vi "1_Power_Transmission_Line_Fault_Classification(Training).vi"() -> ()   [LabVIEW 2020]
uses:
  <vilib>/Ngene/Deep Learning Toolkit/Toolkit/NN_Train/Controls/NN_LR_Policy_Cfg.ctl
  <vilib>/Ngene/Deep Learning Toolkit/Toolkit/NN_Train/Controls/NN_LR_Policy_Type.ctl
  <vilib>/Ngene/Deep Learning Toolkit/Toolkit/NN_Train/Controls/NN_Train_Session_Data.ctl
  <vilib>/Ngene/Deep Learning Toolkit/Toolkit/NN_Train/Controls/NN_Train_Params.ctl
  <vilib>/Ngene/Deep Learning Toolkit/Toolkit/NN_Train/Controls/NN_Train_Optimizer.ctl
  <vilib>/Ngene/Deep Learning Toolkit/Toolkit/NN_Train/Controls/NN_Train_Data_Sampling.ctl
  <vilib>/Ngene/Deep Learning Toolkit/Toolkit/NN_Network/Controls/NN_Device.ctl
  <vilib>/Ngene/Deep Learning Toolkit/Toolkit/NN_Layers/Layers/Input/Controls/NN_Layer_Config(Input1D).ctl
  <vilib>/Ngene/Deep Learning Toolkit/Toolkit/NN_Data/Controls/NN_Data_type.ctl
  <vilib>/Ngene/Deep Learning Toolkit/Toolkit/NN_Layers/Layers/FC/Controls/NN_Layer_Config(FC).ctl
  <vilib>/Ngene/Deep Learning Toolkit/Toolkit/NN_Layers/Layers/BatchNorm/Controls/NN_BN_Params.ctl
  <vilib>/Ngene/Deep Learning Toolkit/Toolkit/NN_Activations/Controls/NN_Activation_Type.ctl
  <vilib>/Ngene/Deep Learning Toolkit/Toolkit/NN_Layers/Controls/NN_Layer_Init_Params.ctl
  <vilib>/Ngene/Deep Learning Toolkit/Toolkit/NN_Layers/Controls/NN_Layer_Weight_Init_Type.ctl
  <vilib>/Ngene/Deep Learning Toolkit/Toolkit/NN_Network/Controls/NN_Save_Before_Destroy_Options.ctl
  <vilib>/Ngene/Deep Learning Toolkit/Toolkit/NN_Layers/Layers/DropOut3D/Controls/NN_Layer_Config(DropOut3D).ctl
  <vilib>/Ngene/Deep Learning Toolkit/Toolkit/NN_Layers/Layers/FC/NN_Layer_Create(FC).vi
  <vilib>/Ngene/Deep Learning Toolkit/Toolkit/NN_Layers/Layers/Dropout/NN_Layer_Create(DropOut).vi
  <vilib>/Ngene/Deep Learning Toolkit/Toolkit/NN_Layers/Layers/Input/NN_Layer_Create(Input1D).vi
  <vilib>/Ngene/Deep Learning Toolkit/Toolkit/NN_Train/Eval_Loss/NN_Calc_Cofusion_Matrix/NN_Calc_Confusion_Matrix(In1D_Out1D).vi
  <vilib>/Ngene/Deep Learning Toolkit/Toolkit/NN_Train/Loss_Functions/NN_Set_Loss(CrossEntropy).vi
  <vilib>/Ngene/Deep Learning Toolkit/Toolkit/NN_Train/Eval_Loss/NN_Eval_Test_Error_Loss/NN_Eval(In1D_Out1D).vi
  <vilib>/Ngene/Deep Learning Toolkit/Toolkit/NN_Network/subVIs/NN_Predict/NN_Predict(In1D_Out1D).vi
  <vilib>/Ngene/Deep Learning Toolkit/Toolkit/NN_Layers/Layers/SoftMax/NN_Layer_Create(SoftMax).vi
  <vilib>/Ngene/Deep Learning Toolkit/Toolkit/Deep_Learning_Toolkit_by_Ngene.lvlib
  <vilib>/ptbypt/NI_PtbyPt.lvlib
panel:
  in  "Tab Control":enum32{"Training", "Evaluation"}(tab)
  in  "LR Update Policy":T1={"Policy_Type"=enum."Step", "LR0"=1e-05, "k"=200.0, "WarmUp_Policy"=enum."Ramp", "WarmUp_Iter"=1000, "WarmUp_Ratio"=10.0} {"WarmUp_Ratio" min=1; "WarmUp_Iter" min=1; "LR0" format="%.7f"}
  out "Session Data":T3={"Epochs"=251.7248, "Tot_Iter"=58998, "LR"=5e-06, "LR_iter"=58999}
  in  "NN_Train_Params":T4={"Optimizer"=enum."Adam", "Beta_1"=0.9, "Beta_2"=0.999, "Weight Decay(L1)"=7e-07, "Weight Decay(L2)"=7e-07, "Data_Sampling"=enum."Random"}
  in  "Stop Training":bool
  out "Test Error":sgl=0.024555556 format="%#.6g"
  out "Test Loss":sgl=0.121348076 format="%#.6g"
  in  "NN_Device":T7=enum."GPU"
  out "Loss Graphs":cluster{"mean":dbl, "mean":dbl, "mean":dbl}(graph)={"mean"=0.14842731654644012, "mean"=0.121348075568676, "mean"=0.02455555647611618}
  in  "Eval":bool
  out "Training Loss":sgl=0.21247883 format="%#.6g"
  in  "Train dataset path":path=path "D:/Ngene/GitHub/deepltk_examples/2_Waveform_Processing/23_Power_Transmission_Line_Fault_Classification/Dataset/Train"
  in  "Test dataset path":path=path "D:/Ngene/GitHub/deepltk_examples/2_Waveform_Processing/23_Power_Transmission_Line_Fault_Classification/Dataset/Test"
  out "Time_Elapsed":dbl=138.95477960000062 format="%<%H:%M:%S>t"
  out "Confusion Matrix":string[][](table)=[["1500", "0", "0", "0", "0", "0", "1.0000"], ["0", "1492", "0", "0", "8", "0", "0.9947"], ["0", "0", "1498", "0", "0", "2", "0.9987"], ["0", "0", "0", "1423", "68", "9", "0.9487"], ["0", "0", "0", "78", "1411", "11", "0.9407"], ["0", "0", "40", "3", "2", "1455", "0.9700"], ["1.0000", "1.0000", "0.9740", "0.9461", "0.9476", "0.9851", ""]]
  # "Overview: This example demonstrates the usage of DeepLTK for solving Power Transmission Line Fault classification problem.\nRequirements: Deep Learning Toolkit for LabVIEW.\nInstructions:\n1.  Run the VI with current configuration of the training parameters and Learning Rate update policy.\n2. Observe how the training loss is decreasing.\n3. Wait about 2 minutes and press the \"Stop\" button when the loss is not decreasing anymore."
  # "Power Transmission Line Fault Classification - Training"
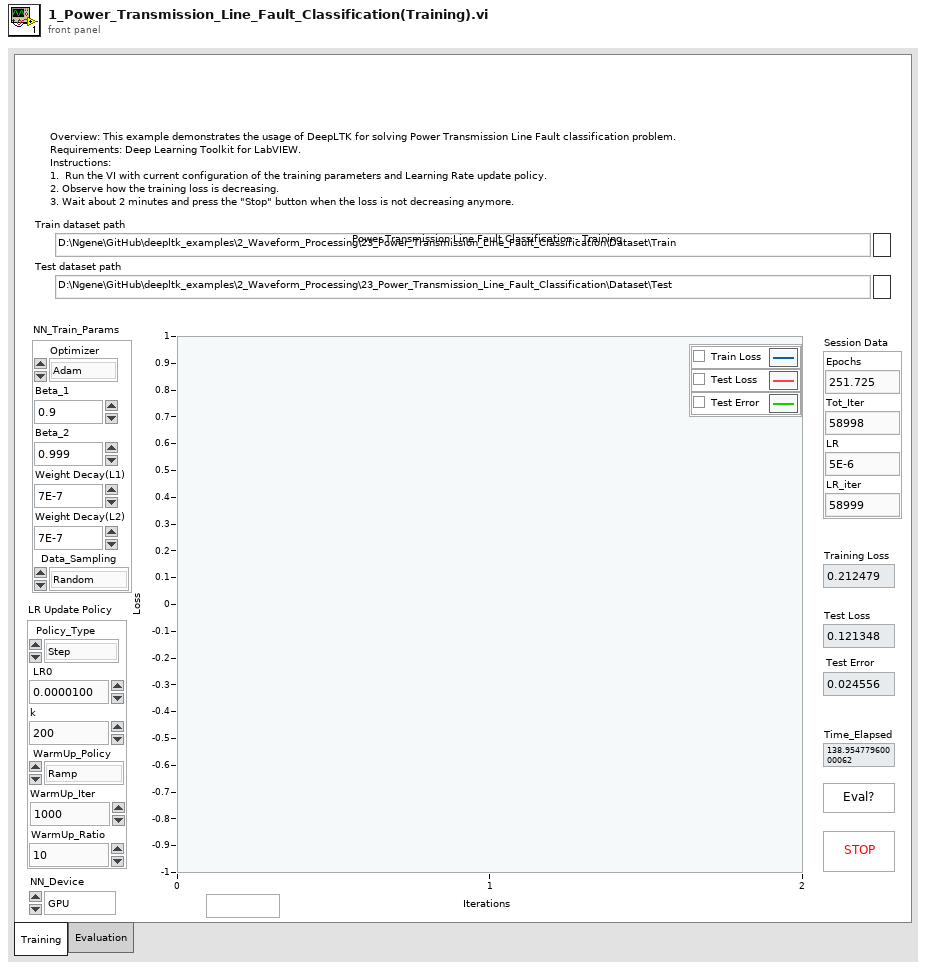
[diagram p1: front panel]
types:
  T1 = typedef "Deep_Learning_Toolkit_by_Ngene.lvlib/NN_LR_Policy_Cfg.ctl" = cluster{"Policy_Type":T2, "LR0":dbl, "k":sgl, "WarmUp_Policy":enum16{"Step", "Ramp"}, "WarmUp_Iter":i32, "WarmUp_Ratio":sgl}
  T2 = typedef "Deep_Learning_Toolkit_by_Ngene.lvlib/NN_LR_Policy_Type.ctl" = enum16{"Manual", "Step", "Exp", "1/t"}
  T3 = typedef "Deep_Learning_Toolkit_by_Ngene.lvlib/NN_Train_Session_Data.ctl" = cluster{"Epochs":sgl, "Tot_Iter":i32, "LR":sgl, "LR_iter":i32}
  T4 = typedef "Deep_Learning_Toolkit_by_Ngene.lvlib/NN_Train_Params.ctl" = cluster{"Optimizer":T5, "Beta_1":sgl, "Beta_2":sgl, "Weight Decay(L1)":sgl, "Weight Decay(L2)":sgl, "Data_Sampling":T6}
  T5 = typedef "Deep_Learning_Toolkit_by_Ngene.lvlib/NN_Train_Optimizer.ctl" = enum16{"SGD", "Adam", "Adagrad", "Adadelta", "RMSProp", "Nesterov"}
  T6 = typedef "Deep_Learning_Toolkit_by_Ngene.lvlib/NN_Train_Data_Sampling.ctl" = enum16{"Random", "Sequential"}
  T7 = typedef "Deep_Learning_Toolkit_by_Ngene.lvlib/NN_Device.ctl" = enum16{"CPU", "GPU"}
  T8 = typedef "Deep_Learning_Toolkit_by_Ngene.lvlib/NN_Layer_Config(DropOut3D).ctl" = cluster{"Name":string, "Probability":sgl}
  T9 = typedef "Deep_Learning_Toolkit_by_Ngene.lvlib/NN_Save_Before_Destroy_Options.ctl" = cluster{"CFG?":bool, "Weights?":bool, "Render?":bool}
  T10 = typedef "Deep_Learning_Toolkit_by_Ngene.lvlib/NN_Layer_Config(FC).ctl" = cluster{"Name":string, "Size":i32, "BN":bool, "BN_Params":T11, "Activation":T12, "Has Bias?":bool, "Init_Params":T13, "Custom_Params":string}
  T11 = typedef "Deep_Learning_Toolkit_by_Ngene.lvlib/NN_BN_Params.ctl" = cluster{"epsilon":sgl, "momentum":sgl}
  T12 = typedef "Deep_Learning_Toolkit_by_Ngene.lvlib/NN_Activation_Type.ctl" = enum16{"Sigmoid", "ReLU", "LReLU", "ReLU6", "GELU", "tanh", "Swish", "Mish", "None"}
  T13 = typedef "Deep_Learning_Toolkit_by_Ngene.lvlib/NN_Layer_Init_Params.ctl" = cluster{"Init_Type":T14, "Value":sgl}
  T14 = typedef "Deep_Learning_Toolkit_by_Ngene.lvlib/NN_Layer_Weight_Init_Type.ctl" = enum16{"Const", "Uniform", "Gaussian", "Xavier"}
  T15 = typedef "Deep_Learning_Toolkit_by_Ngene.lvlib/NN_Layer_Config(Input1D).ctl" = cluster{"Name":string, "Size":i32, "Data_Type":T16, "Shift":sgl, "Scale":sgl}
  T16 = typedef "Deep_Learning_Toolkit_by_Ngene.lvlib/NN_Data_type.ctl" = enum16{"I8", "U8", "I16", "U16", "U32 ARGB", "SGL"}
  T17 = typedef "Deep_Learning_Toolkit_by_Ngene.lvlib/NN_DataSets_All(In1D_Out1D).ctl" = cluster{"Train":T18, "Validation":T18, "Test":T18}
  T18 = typedef "Deep_Learning_Toolkit_by_Ngene.lvlib/NN_DataSet(In1D_Out1D).ctl" = cluster{"Inputs Ref.":variant, "Outputs Ref.":T19, "Dims_In":i32, "Dataset_Size":i32, "Dims_Out":i32, "Labels":string[], "File Paths":path[], "Custom_Data":variant}
  T19 = typedef "Deep_Learning_Toolkit_by_Ngene.lvlib/NN_Data_ref(2D_SGL).ctl" = refnum<data-value>
  T20 = typedef "Deep_Learning_Toolkit_by_Ngene.lvlib/NN.ctl" = cluster{"Name":string, "No of Layers":i32, "mBatch":i32, "Layers":T21[], "Dimty":T22, "Dims_In":T23, "Dims_Out":T23, "Working_Dir":path, "Train?":bool, "Train_Params":T4, "LR_Update_Policy":T1, "Session Data":T3, "Ground_truth":T24, "NNg_hdls":T25, "NN_Device":T7, "GPU Id":i32, "Labels":string[], "Loss_Type":T26, "Loss_Cfg_Prms":variant, "NNG_WS":T27, "DryRun?":bool}
  T21 = typedef "Deep_Learning_Toolkit_by_Ngene.lvlib/NN_Layer_ref.ctl" = refnum<file>
  T22 = typedef "Deep_Learning_Toolkit_by_Ngene.lvlib/NN_In_Out_Dim-ty.ctl" = enum8{"In1D_Out1D", "In3D_Out1D", "In3D_Out3D", "In3D_OutBBox"}
  T23 = typedef "Deep_Learning_Toolkit_by_Ngene.lvlib/NN_Dims(C,H,W).ctl" = cluster{"C":i32, "H":i32, "W":i32}
  T24 = typedef "Deep_Learning_Toolkit_by_Ngene.lvlib/NN_Ground_truth.ctl" = cluster{"Y":variant}
  T25 = typedef "Deep_Learning_Toolkit_by_Ngene.lvlib/nng_cuda_handles.ctl" = cluster{"cudnn":u64, "cublas":u64, "stream":u64, "curand":u64}
  T26 = typedef "Deep_Learning_Toolkit_by_Ngene.lvlib/NN_Loss_Type.ctl" = enum16{"None", "MSE", "CrossEntropy", "YOLO_v2", "YOLO_v4"}
  T27 = typedef "Deep_Learning_Toolkit_by_Ngene.lvlib/NNG_WS.ctl" = cluster{"NNG_WS_Mem":T28, "Max_WS_Size":i64}
  T28 = typedef "Deep_Learning_Toolkit_by_Ngene.lvlib/NNg_WS_Mem_DVR.ctl" = refnum<data-value>
  T29 = typedef "Deep_Learning_Toolkit_by_Ngene.lvlib/NN_Eval_Params.ctl" = cluster{"Loss":sgl, "Error":sgl}
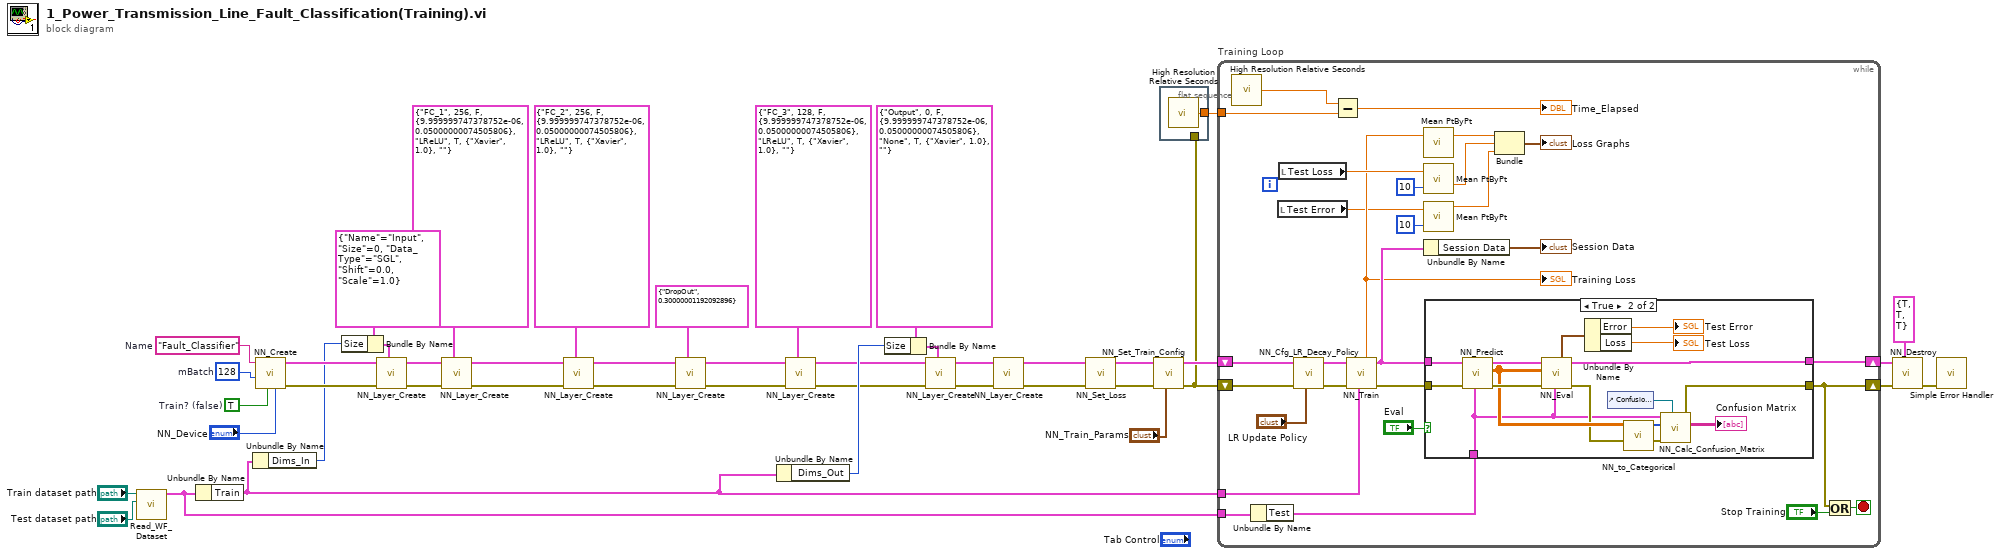
[diagram p0: block diagram]
diagram:
  w27 = "Fault_Classifier"  # Name
  w28 = 128  # mBatch
  w29 = TRUE  # Train? (false)
  n1 = call "Read_WF_Dataset.vi"("Test dataset path"="Test dataset path", "Train dataset path"="Train dataset path") -> ("NN_Dataset"=w11:T17)  [unwired: 9 in]
  n2 = Unbundle By Name(w11) -> ("Train"=w12:T18)
  n3 = Unbundle By Name(w12) -> ("Dims_In"=w13:i32)
  n4 = call <vilib>:"NN_Create.vi"("NN_Device"="NN_Device", "Train? (false)"=w29, "mBatch (1)"=w28, "Name"=w27) -> ("error out"=w43:errorcluster, "NN out"=w44:T20)  [unwired: 6 in]
  n5 = Bundle By Name(cluster=T15 {"Name"="Input", "Size"=0, "Data_Type"=enum."SGL", "Shift"=0.0, "Scale"=1.0} ("Input1D_Cfg"), "Size"=w13) -> (w35:T15)
  n6 = call-poly <vilib>:"NN_Layer_Create.vi"("Input1D_Cfg"=w35, "error in (no error)"=w43, "NN in"=w44) -> ("error out"=w31:errorcluster, "NN out"=w32:T20)  [unwired: 6 in, 1 out]
  n7 = call-poly <vilib>:"NN_Layer_Create.vi"("FC_Cfg"=T10 {"Name"="FC_1", "Size"=256, "BN"=FALSE, "BN_Params"={"epsilon"=1e-05, "momentum"=0.05}, "Activation"=enum."LReLU", "Has Bias?"=TRUE, "Init_Params"={"Init_Type"=enum."Xavier", "Value"=1.0}, "Custom_Params"=""} ("FC_Cfg_1"), "error in (no error)"=w31, "NN in"=w32) -> ("error out"=w2:errorcluster, "NN out"=w3:T20)  [unwired: 6 in, 1 out]
  n8 = call-poly <vilib>:"NN_Layer_Create.vi"("FC_Cfg"=T10 {"Name"="FC_2", "Size"=256, "BN"=FALSE, "BN_Params"={"epsilon"=1e-05, "momentum"=0.05}, "Activation"=enum."LReLU", "Has Bias?"=TRUE, "Init_Params"={"Init_Type"=enum."Xavier", "Value"=1.0}, "Custom_Params"=""} ("FC_Cfg_1"), "error in (no error)"=w2, "NN in"=w3) -> ("error out"=w4:errorcluster, "NN out"=w7:T20)  [unwired: 6 in, 1 out]
  n9 = call-poly <vilib>:"NN_Layer_Create.vi"("DropOut_Cfg"=T8 {"Name"="DropOut", "Probability"=0.3}, "error in (no error)"=w4, "NN in"=w7) -> ("error out"=w5:errorcluster, "NN out"=w6:T20)  [unwired: 6 in, 1 out]
  n10 = Unbundle By Name(w12) -> ("Dims_Out"=w33:i32)
  n11 = call-poly <vilib>:"NN_Layer_Create.vi"("FC_Cfg"=T10 {"Name"="FC_3", "Size"=128, "BN"=FALSE, "BN_Params"={"epsilon"=1e-05, "momentum"=0.05}, "Activation"=enum."LReLU", "Has Bias?"=TRUE, "Init_Params"={"Init_Type"=enum."Xavier", "Value"=1.0}, "Custom_Params"=""} ("FC_Cfg_1"), "error in (no error)"=w5, "NN in"=w6) -> ("error out"=w18:errorcluster, "NN out"=w19:T20)  [unwired: 6 in, 1 out]
  n12 = Bundle By Name(cluster=T10 {"Name"="Output", "Size"=0, "BN"=FALSE, "BN_Params"={"epsilon"=1e-05, "momentum"=0.05}, "Activation"=enum."None", "Has Bias?"=TRUE, "Init_Params"={"Init_Type"=enum."Xavier", "Value"=1.0}, "Custom_Params"=""} ("FC_Cfg_1"), "Size"=w33) -> (w34:T10)
  n13 = call-poly <vilib>:"NN_Layer_Create.vi"("FC_Cfg"=w34, "error in (no error)"=w18, "NN in"=w19) -> ("error out"=w38:errorcluster, "NN out"=w39:T20)  [unwired: 6 in, 1 out]
  n14 = call-poly <vilib>:"NN_Layer_Create.vi"("error in (no error)"=w38, "NN in"=w39) -> ("error out"=w24:errorcluster, "NN out"=w40:T20)  [unwired: 7 in, 1 out]
  n15 = call-poly <vilib>:"NN_Set_Loss.vi"("error in (no error)"=w24, "NN in"=w40) -> ("error out"=w23:errorcluster, "NN out"=w25:T20)  [unwired: 8 in]
  n16 = call <vilib>:"NN_Set_Train_Config.vi"("NN_Train_Params"="NN_Train_Params", "error in (no error)"=w23, "NN in"=w25) -> ("error out"=w9:errorcluster, "NN out"=w30:T20)  [unwired: 7 in]
  n17 = flat-sequence {
    tunnel: w9 -> [_]
    tunnel: [w45] -> w8
    frame #0 {
      n18 = call <vilib>:"High Resolution Relative Seconds.vi"() -> ("relative seconds"=w45:dbl)
    }
  }
  n19 = while "Training Loop" {
    shift-right: [w58] -> w16
    shift-left: w9 -> [w68]
    shift-right: [w64] -> w17
    shift-left: w30 -> [w71]
    tunnel: w12 -> [w53]
    tunnel: w11 -> [w54]
    tunnel: w8 -> [w51]
    stop <- w59 stop-if-true
    n20 = call <vilib>:"High Resolution Relative Seconds.vi"() -> ("relative seconds"=w50:dbl)
    n21 = Unbundle By Name(w54) -> ("Test"=w52:T18)
    n22 = local read "Test Error"() -> (w47:sgl)
    n23 = local read "Test Loss"() -> (w62:sgl)
    n24 = call <vilib>:"NN_Cfg_LR_Decay_Policy.vi"("LR_Decay_Params"="LR Update Policy", "error in (no error)"=w68, "NN in"=w71) -> ("error out"=w69:errorcluster, "NN out"=w70:T20)  [unwired: 7 in]
    n25 = Subtract(x=w50, y=w51) -> (x-y=→"Time_Elapsed":dbl)
    n26 = call <vilib>:"NN_Train.vi"("Train Dataset"=w53, "error in (no error)"=w69, "NN in"=w70) -> ("error out"=w65:errorcluster, "NN out"=w66:T20, "Loss"=w60:sgl)  [unwired: 3 in, 3 out]
    "Training Loss" <- w60
    n27 = call <vilib>:"Mean PtByPt.vi"("x"=w60) -> ("mean"=w56:dbl)  [unwired: 3 in, 1 out]
    n28 = call <vilib>:"Mean PtByPt.vi"("x"=w62, "sample length"=10) -> ("mean"=w57:dbl)  [unwired: 2 in, 1 out]
    n29 = call <vilib>:"Mean PtByPt.vi"("x"=w47, "sample length"=10) -> ("mean"=w46:dbl)  [unwired: 2 in, 1 out]
    n30 = Unbundle By Name(w66) -> ("Session Data"=→"Session Data":T3)
    n31 = case shown="True" "Eval" {
      tunnel: w66 -> [w75 w89]
      tunnel: w65 -> [w74 w88]
      tunnel: [w75 w87] -> w64
      tunnel: [w74 w82] -> w58
      tunnel: w52 -> [_ w79]
      frame False {
      }
      frame True {
        n32 = call-poly <vilib>:"NN_Predict.vi"("Dataset"=w79, "error in (no error)"=w88, "NN in"=w89) -> ("error out"=w90:errorcluster, "Predictions"=w85:sgl[][], "NN out"=w86:T20)  [unwired: 6 in]
        n33 = call-poly <vilib>:"NN_Eval.vi"("Dataset"=w79, "error in (no error)"=w90, "Predictions"=w85, "NN in"=w86) -> ("error out"=w83:errorcluster, "NN out"=w87:T20, "NN_Eval_Params"=w78:T29)  [unwired: 4 in, 1 out]
        n34 = Unbundle By Name(w78) -> ("Error"=→"Test Error":sgl, "Loss"=→"Test Loss":sgl)
        n35 = control-ref of="Confusion Matrix"() -> (w80:refnum<vi>)
        n36 = call <vilib>:"NN_to_Categorical.vi"("Prediction"=w85) -> ("Label_Idx"=w84:i32[])  [unwired: 10 in]
        n37 = call-poly <vilib>:"NN_Calc_Confusion_Matrix.vi"("Confusion Matrix (Table) ref."=w80, "error in (no error)"=w83, "Predictions"=w84, "Dataset"=w79) -> ("error out"=w82:errorcluster, "Confusion Matrix (Table)"=→"Confusion Matrix":string[][])  [unwired: 3 in, 3 out]
      }
    }
    n38 = Bundle("mean"=w56, "mean"=w57, "mean"=w46) -> (→"Loss Graphs":cluster{"mean":dbl, "mean":dbl, "mean":dbl})  [unwired: 1 in]
    n39 = Or(x=w58, y="Stop Training") -> (x .or. y?=w59:bool)
  }
  n40 = call <vilib>:"NN_Destroy.vi"("Save (T, T, T)"=T9 {"CFG?"=TRUE, "Weights?"=TRUE, "Render?"=TRUE}, "error in (no error)"=w16, "NN in"=w17) -> ("error out"=w37:errorcluster)  [unwired: 7 in, 1 out]
  n41 = call <vilib>:"Simple Error Handler.vi"("error in (no error)"=w37) -> ()  [unwired: 4 in, 5 out]
